vi "test2-DifferentChainNodesProcessDifferentAllowedMessages.vi"(8 "error in (no error)":errorcluster, 11 "TestCase in":refnum<class "testcase-CSMChainMode.lvclass">) -> (0 "error out":errorcluster, 3 "TestCase out":refnum<class "testcase-CSMChainMode.lvclass">)   [LabVIEW 2017, in "testcase-CSMChainMode.lvclass"]
uses:
  testcase-CSMChainMode.lvclass
  <vilib>/addons/_JKI Toolkits/VI Tester/TestCase.llb/TestCase.lvclass
  src/user.lib/_NEVSTOP/Communicable State Machine(CSM)/Communicable State Machine.lvlib
  C:/Program Files (x86)/National Instruments/LabVIEW 2017/vi.lib/addons/_JKI Toolkits/VI Tester/TestCase.llb/TestCase.lvclass
panel:
  out "LoopCount":i32
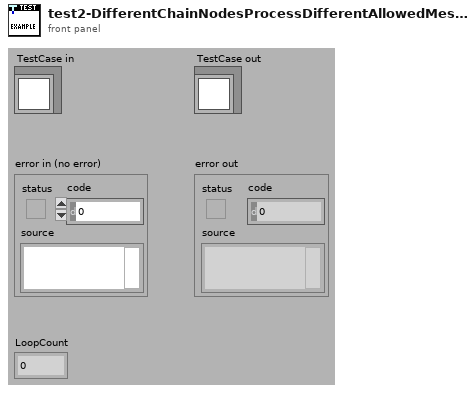
[diagram p1: front panel]
types:
  T1 = cluster{"Allowed":string, "Not Allowed":string[]}[]
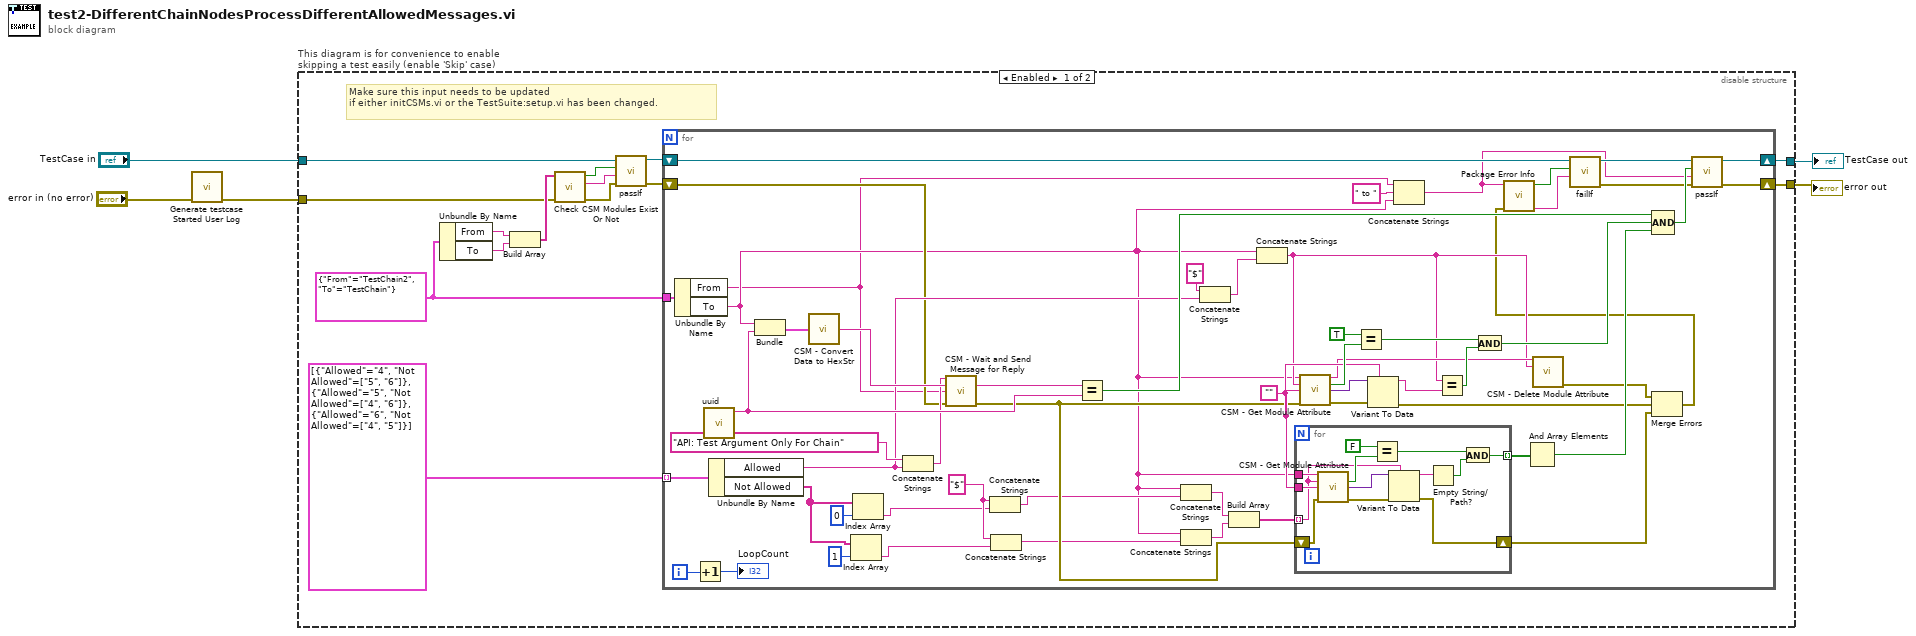
[diagram p0: block diagram]
diagram:
  n1 = call "Generate testcase Started User Log.vi"("Error In"="error in (no error)") -> ("error out"=w1:errorcluster)  [unwired: 10 in]
  n2 = disable-structure "This diagram is for convenience to enable skipping a test easily (enable 'Skip' case)" shown="Enabled" {
    disable-tunnel: "TestCase in" -> [w10 w92]
    disable-tunnel: [w19 w90] -> w2
    disable-tunnel: [w18 w91] -> w4
    disable-tunnel: w1 -> [w8 w89]
    frame Enabled {
      w6 = cluster{"From":string, "To":string} {"From"="TestChain2", "To"="TestChain"} ("Cluster")
      # "Make sure this input needs to be updated \nif either initCSMs.vi or the TestSuite:setup.vi has been changed."
      n3 = Unbundle By Name(w6) -> ("From"=w12:string, "To"=w13:string)
      n4 = Build Array(w12, w13) -> (w11:string[])
      n5 = call "Check CSM Modules Exist Or Not.vi"("error in"=w8, "CSM names in"=w11) -> ("error out"=w14:errorcluster, "Debug string"=w15:string, "All Modules Exist?"=w16:bool)  [unwired: 7 in]
      n6 = call-dynamic "passIf.vi"("error in (no error)"=w14, "message (\"\")"=w15, "pass"=w16, "TestCase in"=w10) -> ("error out"=w7:errorcluster, "TestCase out"=w9:refnum<class "testcase-CSMChainMode.lvclass">)  [unwired: 6 in]
      n7 = for {
        tunnel: w6 -> [w75]
        shift-right: [w70] -> w19
        shift-left: w9 -> [w26]
        shift-right: [w69] -> w18
        shift-left: w7 -> [w30]
        tunnel: T1 [{"Allowed"="4", "Not Allowed"=["5", "6"]}, {"Allowed"="5", "Not Allowed"=["4", "6"]}, {"Allowed"="6", "Not Allowed"=["4", "5"]}] -> [w47] mode=indexing
        i -> [w49]
        w41 = "$" ("string")
        w58 = ""
        n8 = Unbundle By Name(w75) -> ("From"=w21:string, "To"=w22:string)
        n9 = Increment(x=w49) -> (x+1=→"LoopCount":i32)
        n10 = call "uuid.vi"() -> ("UUID"=w61:string)  [unwired: 11 in]
        n11 = Unbundle By Name(w47) -> ("Allowed"=w43:string, "Not Allowed"=w37:string[])
        n12 = Bundle("To"=w22, "UUID"=w61) -> (w74:cluster{"To":string, "UUID":string})  [unwired: 1 in]
        n13 = call "CSM - Convert Data to HexStr.vi"("Variant"=w74) -> ("HEX String (0-9,A-F)"=w73:string)  [unwired: 8 in]
        n14 = Index Array(array=w37, index=1) -> (element=w36:string)
        n15 = Index Array(array=w37, index=0) -> (element=w39:string)
        n16 = Concatenate Strings("API: Test Argument Only For Chain" ("State"), w43) -> (w45:string)
        n17 = call "CSM - Wait and Send Message for Reply.vi"("State"=w45, "Arguments (\"\")"=w73, "Target Module"=w21, "Error In (No Error)"=w30) -> ("Response"=w62:string, "error out"=w52:errorcluster)  [unwired: 8 in, 2 out]
        n18 = Concatenate Strings(w41, w39) -> (w35:string)
        n19 = Concatenate Strings(w41, w36) -> (w34:string)
        n20 = Equal?(x=w62, y=w61) -> (x = y?=w72:bool)
        n21 = Concatenate Strings(w22, w35) -> (w57:string)
        n22 = Concatenate Strings(w22, w34) -> (w56:string)
        n23 = Concatenate Strings("$" ("string"), w43) -> (w42:string)
        n24 = Build Array(w57, w56) -> (w55:string[])
        n25 = Concatenate Strings(w22, w42) -> (w32:string)
        n26 = for {
          tunnel: w58 -> [w88]
          tunnel: w22 -> [w83]
          tunnel: w55 -> [w82] mode=indexing
          tunnel: [w78] -> w54 mode=indexing
          shift-right: [w76] -> w50
          shift-left: w52 -> [w77]
          n27 = call "CSM - Get Module Attribute.vi"("CSM Name"=w83, "Attribute"=w82, "Default Value (Empty Variant)"=w88, "Error In"=w77) -> ("Found"=w85:bool, "Value"=w86:variant, "error out"=w87:errorcluster)  [unwired: 7 in, 2 out]
          n28 = Equal?(x=FALSE, y=w85) -> (x = y?=w79:bool)
          n29 = Variant To Data(error in=w87, type=w82, Variant=w86) -> (data=w81:string, error out=w76:errorcluster)
          n30 = Empty String/Path?(string/path=w81) -> (empty?=w80:bool)
          n31 = And(x=w79, y=w80) -> (x .and. y?=w78:bool)
        }
        n32 = call "CSM - Get Module Attribute.vi"("CSM Name"=w22, "Attribute"=w32, "Default Value (Empty Variant)"=w58, "Error In"=w52) -> ("CSM Name (Dup)"=w33:string, "Found"=w68:bool, "Value"=w65:variant, "error out"=w66:errorcluster)  [unwired: 7 in, 1 out]
        n33 = Equal?(x=TRUE, y=w68) -> (x = y?=w64:bool)
        n34 = Variant To Data(error in=w66, type=w58, Variant=w65) -> (data=w60:string, error out=w51:errorcluster)
        n35 = Concatenate Strings(w21, " to " ("string"), w22) -> (w20:string)
        n36 = Equal?(x=w32, y=w60) -> (x = y?=w63:bool)
        n37 = And(x=w64, y=w63) -> (x .and. y?=w59:bool)
        n38 = And Array Elements(Boolean array=w54) -> (logical AND=w53:bool)
        n39 = call "CSM - Delete Module Attribute.vi"("CSM Name"=w33, "Attribute"=w32) -> ("error out"=w31:errorcluster)  [unwired: 10 in, 3 out]
        n40 = Compound Arithmetic op=AND(w72, w59, w53) -> (w71:bool)
        n41 = Merge Errors(w31, w51, w50) -> (w23:errorcluster)
        n42 = call "Package Error Info.vi"("error in"=w23, "String in"=w20) -> ("packed error info out"=w28:string, "error status"=w29:bool)  [unwired: 8 in]
        n43 = call-dynamic "failIf.vi"("message (\"\")"=w28, "fail"=w29, "TestCase in"=w26) -> ("error out"=w24:errorcluster, "TestCase out"=w25:refnum<class "testcase-CSMChainMode.lvclass">)  [unwired: 7 in]
        n44 = call-dynamic "passIf.vi"("error in (no error)"=w24, "message (\"\")"=w20, "pass"=w71, "TestCase in"=w25) -> ("error out"=w69:errorcluster, "TestCase out"=w70:refnum<class "testcase-CSMChainMode.lvclass">)  [unwired: 6 in]
      }
    }
    frame Disabled {
      # "skip test result while test is under development"
      n45 = call <vilib>:"skip.vi"("error in (no error)"=w89, "TestCase in"=w92) -> ("error out"=w91:errorcluster, "TestCase out"=w90:refnum<class "testcase-CSMChainMode.lvclass">)  [unwired: 8 in]
    }
  }
  "error out" <- w4
  "TestCase out" <- w2
